vi "close.vi"(8 "error in (no error)":errorcluster, 11 "USB-6001 in":refnum<class "USB-6001.lvclass">) -> (0 "error out":errorcluster, 3 "USB-6001 out":refnum<class "USB-6001.lvclass">)   [LabVIEW 2025, in "USB IO.lvlib" / "USB-6001.lvclass"]
uses:
  USB-6001.lvclass
  USB-6001.lvclass/USB-6001.ctl
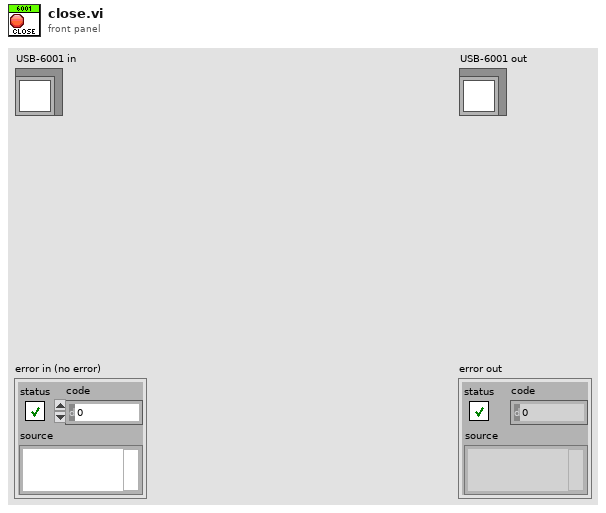
[diagram p1: front panel]
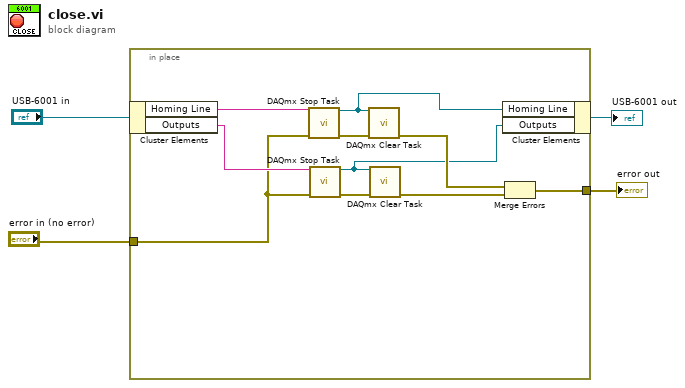
[diagram p0: block diagram]
diagram:
  n1 = in-place {
    in-place-border: "error in (no error)" -> [w10]
    in-place-border: [w7] -> w1
    n2 = in-place-cluster #1("USB-6001 in") -> ("Homing Line"=w14:string, "Outputs"=w11:string)
    n3 = call <vilib>:"DAQmx Stop Task.vi"("task/channels in"=w14, "error in"=w10) -> ("task out"=w6:refnum<k21>, "error out"=w13:errorcluster)  [unwired: 12 in]
    n4 = call <vilib>:"DAQmx Stop Task.vi"("task/channels in"=w11, "error in"=w10) -> ("task out"=w5:refnum<k21>, "error out"=w12:errorcluster)  [unwired: 12 in]
    n5 = call <vilib>:"DAQmx Clear Task.vi"("task in"=w6, "error in"=w13) -> ("error out"=w9:errorcluster)  [unwired: 13 in]
    n6 = call <vilib>:"DAQmx Clear Task.vi"("task in"=w5, "error in"=w12) -> ("error out"=w8:errorcluster)  [unwired: 13 in]
    n7 = in-place-cluster #1("Homing Line"=w6, "Outputs"=w5) -> (→"USB-6001 out":refnum<class "USB-6001.lvclass">)
    n8 = Merge Errors(w9, w8) -> (w7:errorcluster)
  }
  "error out" <- w1
